vi "Exo_discriminant_boite_de_calcul.vi"() -> ()   [LabVIEW 2012]
panel:
  out "output variable":dbl
  in  "c":dbl
  in  "a":dbl
  in  "b":dbl
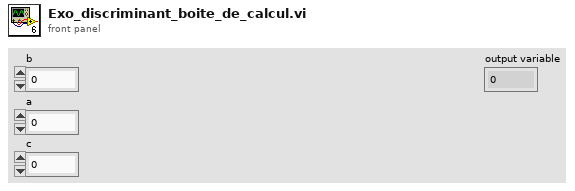
[diagram p1: front panel]
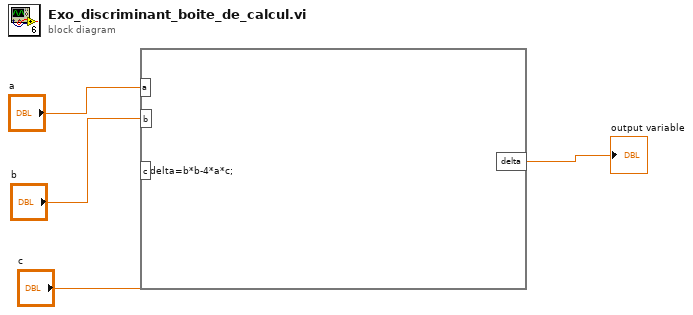
[diagram p0: block diagram]
diagram:
  n1 = formula code="delta=b*b-4*a*c;"("c"="c", "b"="b", "a"="a") -> ("delta"=→"output variable":dbl)
